vi "from string.vi"(8 "error in":errorcluster, 9 "data":string, 10 "version":string, 11 "fixed channel configuration in":refnum<class "control module configuration.lvclass">=refnum) -> (0 "error out":errorcluster, 3 "fixed channel configuration out":refnum<class "control module configuration.lvclass">)   [LabVIEW 2014, in "control module configuration.lvclass"]
doc: "Provides an interface for loading a module configuration from a file or other serialized data source. It is recommended that all children of this class store data in two sets--data required for its own initialization, and any data required for parent initialization--and that each implementation uses the <b>Call Parent Method</b> primitive to de-serialize parent information. As a result, it is expected that every module configuration class calls <b>component configuration.lvclass:From String.vi</b>.\nNI Tag Bus Module Framework 1.0.3.43\nNI Systems Engineering"
uses:
  control module configuration.lvclass
  <vilib>/NI/Tag Bus Module Framework/channel/TBM channel.lvclass
  <vilib>/NI/Configuration Framework/serializable configuration/NISE_CEF_serializable configuration.lvclass
  <vilib>/NI/Tag Bus Module Framework/runtime/error classification.ctl
  error classification setting.ctl
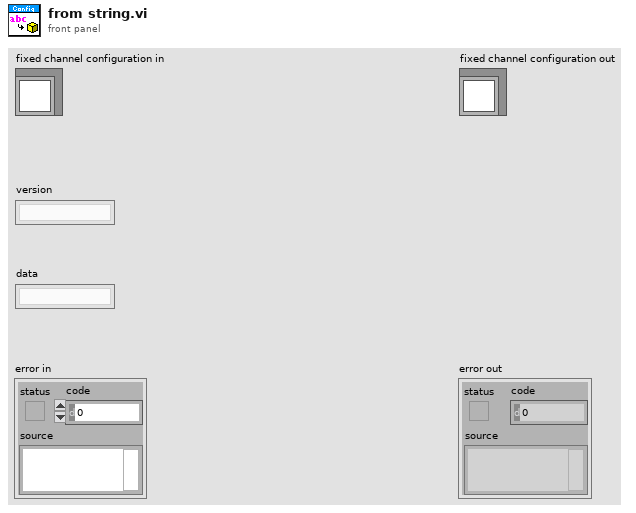
[diagram p1: front panel]
types:
  T1 = typedef "control module configuration.lvclass/error classification setting.ctl" = cluster{"code":i32, "error classification":T2}
  T2 = typedef "TBM module execution interface.lvclass/error classification.ctl" = enum16{"unknown", "none", "trivial", "recoverable", "critical"}
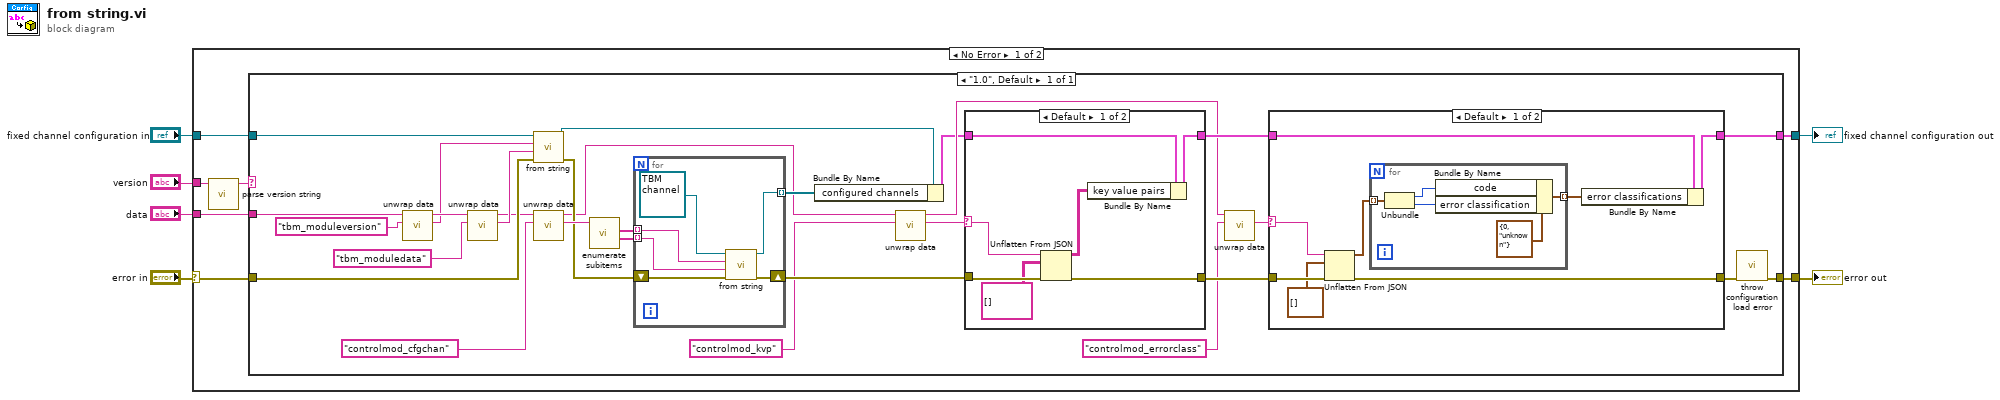
[diagram p0: block diagram]
diagram:
  n1 = case shown="No Error" "error in" {
    selector: "error in" -> [w7 w74]
    tunnel: "data" -> [w13 _]
    tunnel: "fixed channel configuration in" -> [w12 w73]
    tunnel: [w11 w73] -> w5
    tunnel: [w10 w74] -> w4
    tunnel: "version" -> [w9 _]
    frame No Error {
      n2 = call <vilib>:"parse version string.vi"("full version"=w9) -> ("major.minor version"=w8:string)  [unwired: 7 in, 3 out]
      n3 = case shown="\"1.0\", Default" w8 {
        tunnel: w13 -> [w38]
        tunnel: w7 -> [w40]
        tunnel: w12 -> [w42]
        tunnel: [w39] -> w11
        tunnel: [w41] -> w10
        frame "1.0", Default {
          n4 = call <vilib>:"unwrap data.vi"("identifier"="tbm_moduleversion" ("additional identifier"), "data to unwrap"=w38) -> ("unwrapped data"=w32:string, "remaining string"=w34:string)  [unwired: 8 in]
          n5 = call <vilib>:"unwrap data.vi"("identifier"="tbm_moduledata" ("additional identifier"), "data to unwrap"=w34) -> ("unwrapped data"=w33:string, "remaining string"=w31:string)  [unwired: 8 in]
          n6 = call-parent "from string.vi"("error in"=w40, "data"=w33, "version"=w32, "module configuration in"=w42) -> ("error out"=w29:errorcluster, "module configuration out"=w37:refnum<class "control module configuration.lvclass">)  [unwired: 6 in]
          n7 = call <vilib>:"unwrap data.vi"("identifier"="controlmod_cfgchan", "data to unwrap"=w31) -> ("unwrapped data"=w30:string, "remaining string"=w25:string)  [unwired: 8 in]
          n8 = call <vilib>:"enumerate subitems.vi"("data to enumerate"=w30) -> ("associated data"=w27:string[], "discovered subitems"=w28:string[])  [unwired: 8 in, 1 out]
          n9 = for {
            shift-right: [w72] -> w24
            shift-left: w29 -> [w71]
            tunnel: w28 -> [w69] mode=indexing
            tunnel: w27 -> [w68] mode=indexing
            tunnel: [w70] -> w26 mode=indexing
            n10 = call-dynamic "from string.vi"("error in"=w71, "channel data"=w68, "identifier"=w69, "channel in"=refnum<class "TBM channel.lvclass"> refnum) -> ("error out"=w72:errorcluster, "channel out"=w70:refnum<class "TBM channel.lvclass">)  [unwired: 6 in]
          }
          n11 = Bundle By Name(cluster=w37, "configured channels"=w26) -> (w14:cluster{})
          n12 = call <vilib>:"unwrap data.vi"("identifier"="controlmod_kvp", "data to unwrap"=w25) -> ("unwrapped data"=w23:string, "remaining string"=w18:string)  [unwired: 8 in]
          n13 = case shown="Default" w23 {
            selector: w23 -> [w61 _]
            tunnel: w24 -> [w63 w66]
            tunnel: [w62 w66] -> w22
            tunnel: w14 -> [w64 w65]
            tunnel: [w58 w65] -> w20
            frame Default {
              n14 = Unflatten From JSON(JSON string=w61, type and defaults=string[][] [] ("key value pairs"), error in (no error)=w63) -> (value=w60:string[][], error out=w62:errorcluster)  [unwired: 4 in]
              n15 = Bundle By Name(cluster=w64, "key value pairs"=w60) -> (w58:cluster{})
            }
            frame "" {
            }
          }
          n16 = call <vilib>:"unwrap data.vi"("identifier"="controlmod_errorclass", "data to unwrap"=w18) -> ("unwrapped data"=w19:string)  [unwired: 8 in, 1 out]
          n17 = case shown="Default" w19 {
            selector: w19 -> [w47 _]
            tunnel: w22 -> [w49 w57]
            tunnel: [w48 w57] -> w21
            tunnel: w20 -> [w50 w56]
            tunnel: [w45 w56] -> w39
            frame Default {
              n18 = Unflatten From JSON(JSON string=w47, type and defaults=cluster{i32, i32}[] [], error in (no error)=w49) -> (value=w44:cluster{i32, i32}[], error out=w48:errorcluster)  [unwired: 4 in]
              n19 = for {
                tunnel: w44 -> [w55] mode=indexing
                tunnel: [w51] -> w43 mode=indexing
                n20 = Unbundle(w55) -> (w53:i32, w52:i32)
                n21 = Bundle By Name(cluster=T1 {"code"=0, "error classification"=enum."unknown"} ("error classification"), "code"=w53, "error classification"=w52) -> (w51:T1)
              }
              n22 = Bundle By Name(cluster=w50, "error classifications"=w43) -> (w45:cluster{})
            }
            frame "" {
            }
          }
          n23 = call <vilib>:"throw configuration load error.vi"("error in"=w21) -> ("error out"=w41:errorcluster)  [unwired: 10 in]
        }
      }
    }
    frame Error {
    }
  }
  "error out" <- w4
  "fixed channel configuration out" <- w5
